vi "Write Fetch Interval.vi"(8 "error in (no error)":errorcluster, 10 "Fetch Interval":i32, 11 "ETS_EM2090 in":refnum<class "ETS_EM2090.lvclass">) -> (0 "error out":errorcluster, 3 "ETS_EM2090 out":refnum<class "ETS_EM2090.lvclass">)   [LabVIEW 2023, in "Turn Table and Mast.lvlib" / "ETS_EM2090.lvclass"]
uses:
  ETS_EM2090.lvclass
  ETS_EM2090.lvclass/ETS_EM2090.ctl
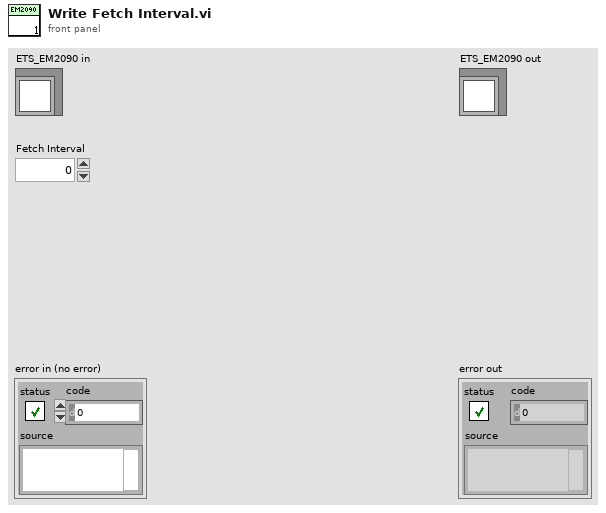
[diagram p1: front panel]
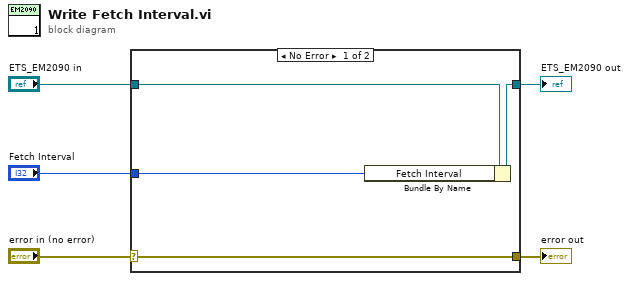
[diagram p0: block diagram]
diagram:
  n1 = case shown="No Error" "error in (no error)" {
    selector: "error in (no error)" -> [w9 w10]
    tunnel: [w9 w10] -> w4
    tunnel: [w7 w11] -> w2
    tunnel: "ETS_EM2090 in" -> [w8 w11]
    tunnel: "Fetch Interval" -> [w6 _]
    frame No Error {
      n2 = Bundle By Name(cluster=w8, "Fetch Interval"=w6) -> (w7:refnum<class "ETS_EM2090.lvclass">)
    }
    frame Error {
    }
  }
  "error out" <- w4
  "ETS_EM2090 out" <- w2
